vi "XNET.Create.Frame.vi"(8 "error in":errorcluster, 10 "CAN Frame":T1={"Frame name"="frame1", "Identifier"=1, "Payload Length"=8, "Timing Type"=1, "Transmit Time"=0.0, "Extended Identifier?"=FALSE, "Comment"="", "IO Mode"=0} {"IO Mode" items=["CAN 2.0", "CAN FD", "CAN FD+BRS"]; "Timing Type" items=["Cyclic Data", "Event Data", "Cyclic Remote", "Event Remote"]}, 11 "cluster in":refnum<k21>) -> (0 "error out":errorcluster, 2 "frame out":refnum<k21>, 3 "cluster out":refnum<k21>)   [LabVIEW 2024, in "Diagnostics Addon Shared.lvlib"]
uses:
  Diagnostics Addon Shared.lvlib
  Types/XNET.Frame.ctl
  <vilib>/xnet/xnet.llb/XNET Database Create (Frame).vi
  <resource>/objmgr/xnet.rc
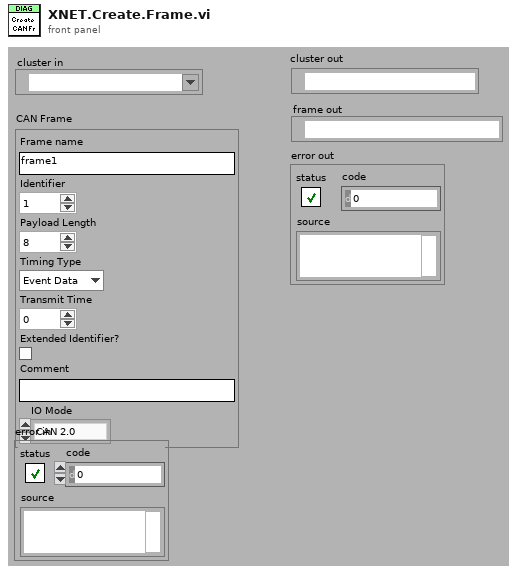
[diagram p1: front panel]
types:
  T1 = typedef "Diagnostics Addon Shared.lvlib/XNET.Frame.ctl" = cluster{"Frame name":string, "Identifier":u32, "Payload Length":u32, "Timing Type":u32, "Transmit Time":dbl, "Extended Identifier?":bool, "Comment":string, "IO Mode":u32}
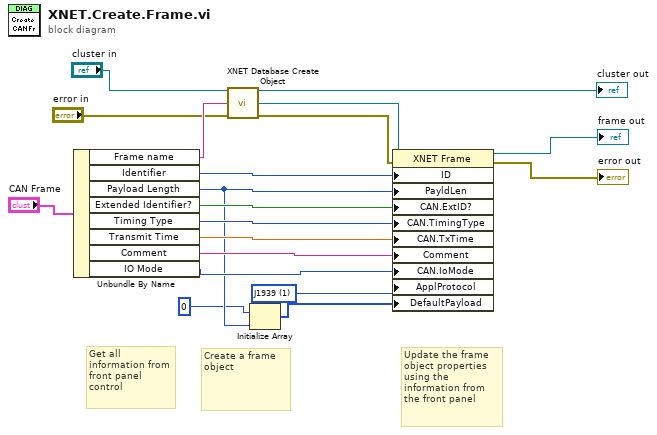
[diagram p0: block diagram]
diagram:
  w5 = u32 1 items=["None", "J1939"] ("Application Protocol")
  # "Update the frame object properties using the information from the front panel"
  # "Create a frame object"
  # "Get all information from front panel control"
  n1 = Unbundle By Name("CAN Frame") -> ("Frame name"=w15:string, "Identifier"=w16:u32, "Payload Length"=w3:u32, "Extended Identifier?"=w17:bool, "Timing Type"=w18:u32, "Transmit Time"=w19:dbl, "Comment"=w7:string, "IO Mode"=w4:u32)
  n2 = call-poly <vilib>:"XNET Database Create Object.vi"("cluster in"="cluster in", "frame name"=w15, "error in (no error)"="error in") -> ("cluster out"=→"cluster out":refnum<k21>, "frame out"=w8:refnum<k21>, "error out"=w9:errorcluster)  [unwired: 10 in]
  n3 = Initialize Array(u8 0, w3) -> (w1:u8[])
  n4 = property class="XNET Frame"(reference=w8, error in=w9, "ID"=w16, "PayldLen"=w3, "CAN.ExtID?"=w17, "CAN.TimingType"=w18, "CAN.TxTime"=w19, "Comment"=w7, "CAN.IoMode"=w4, "ApplProtocol"=w5, "DefaultPayload"=w1) -> (reference out=→"frame out":refnum<k21>, error out=→"error out":errorcluster)
